vi "PicoScope4000ExampleStreaming.vi"() -> ()   [LabVIEW 2010]
doc: "This example demonstrates how to use the PicoScope Labview library to stream data from a PicoScope 4000 Series Device"
uses:
  PicoScope4000Lib/PicoScope4000AnalogChannelSettingsIEPE.ctl
  PicoScope4000Lib/PicoScope4000Buffer and Transfer Settings.ctl
panel:
  in  "Write TDMS":bool
  in  "Channel B Settings":T1={"Enabled"=FALSE, "Range"=6, "Bandwidth Limit"=0, "Coupling"=1} {"Coupling" items=["AC", "DC", "IEPE"]; "Bandwidth Limit" items=["Off", "200kHz"]; "Range" items=["10 mV", "20 mV", "50 mV", "100 mV", "200 mV", "500 mV", "1 V", "2 V", "5 V", "10 V", "20 V", "50 V ", "100 V"]}
  out "Unit Info":T2
  in  "Channel A Settings":T1={"Enabled"=TRUE, "Range"=6, "Bandwidth Limit"=0, "Coupling"=1} {"Coupling" items=["AC", "DC", "IEPE"]; "Bandwidth Limit" items=["Off", "200kHz"]; "Range" items=["10 mV", "20 mV", "50 mV", "100 mV", "200 mV", "500 mV", "1 V", "2 V", "5 V", "10 V", "20 V", "50 V ", "100 V"]}
  out "Analog Channels":cluster{i32, dbl, "Data (Volts)":dbl[]}[](graph)=[{0, 8e-09, "Data (Volts)"=[]}, {0, 8e-09, "Data (Volts)"=[]}, {0, 8e-09, "Data (Volts)"=[]}, {0, 8e-09, "Data (Volts)"=[]}, {0, 8e-09, "Data (Volts)"=[]}, {0, 8e-09, "Data (Volts)"=[]}, {0, 8e-09, "Data (Volts)"=[]}, {0, 8e-09, "Data (Volts)"=[]}]
  out "Raw Sample Interval (sec)":dbl format="%#.5p"
  out "Max ADC value":i16
  out "Chunk time(ms)":u32
  out "Elapsed time":dbl
  in  "Data file":path=path "PicoScope4000aExampleStreaming Data"
  out "size(s)":i32
  out "Queue depth":i32(graph)
  out "queue depth":i32
  in  "Buffer and Transfer Settings":T3={"startIndex"=0, "Samples"=1000000, "Down Sample Ratio"=1, "Down-Sample Mode"=0} {"Down-Sample Mode" items=["None", "Aggregate", "Average"]; "Down Sample Ratio" step=1; "Samples" format="%_6p"}
  out "TriggeredAt (In Buffer)":u32 format="%#.6p"
  out "TriggeredAt (Total samples)":u32 format="%#.6p"
  in  "Acquisition Settings":T4={"Auto Stop"=TRUE, "Desired Sample Interval"=1, "Pre-trigger Samples"=0, "Post-trigger Samples"=1000000, "Down-Sample Ratio"=1, "Down-Sample Mode"=0, "Time Units"=3} {"Time Units" items=["Nanoseconds (ns)"=2, "Microseconds (us)"=3, "Milliseconds (ms)"=4, "Seconds (s)"=5]; "Down-Sample Mode" items=["None"=0, "Aggregate"=1, "Decimate"=2, "Average"=4]; "Post-trigger Samples" format="%#.6p"; "Pre-trigger Samples" format="%#_6p"}
  out "Triggered":bool
  out "DownSample Interval (sec)":dbl format="%#.5p"
  out "Total Samples":u32 format="%#.6p"
  out "Auto Stopped":bool
  in  "Serial Number":string
  in  "Open Using Serial Number":bool
  out "Number of Samples per Capture":u32 format="%#.6p"
  in  "Apply Settings":bool
  in  "stop":bool
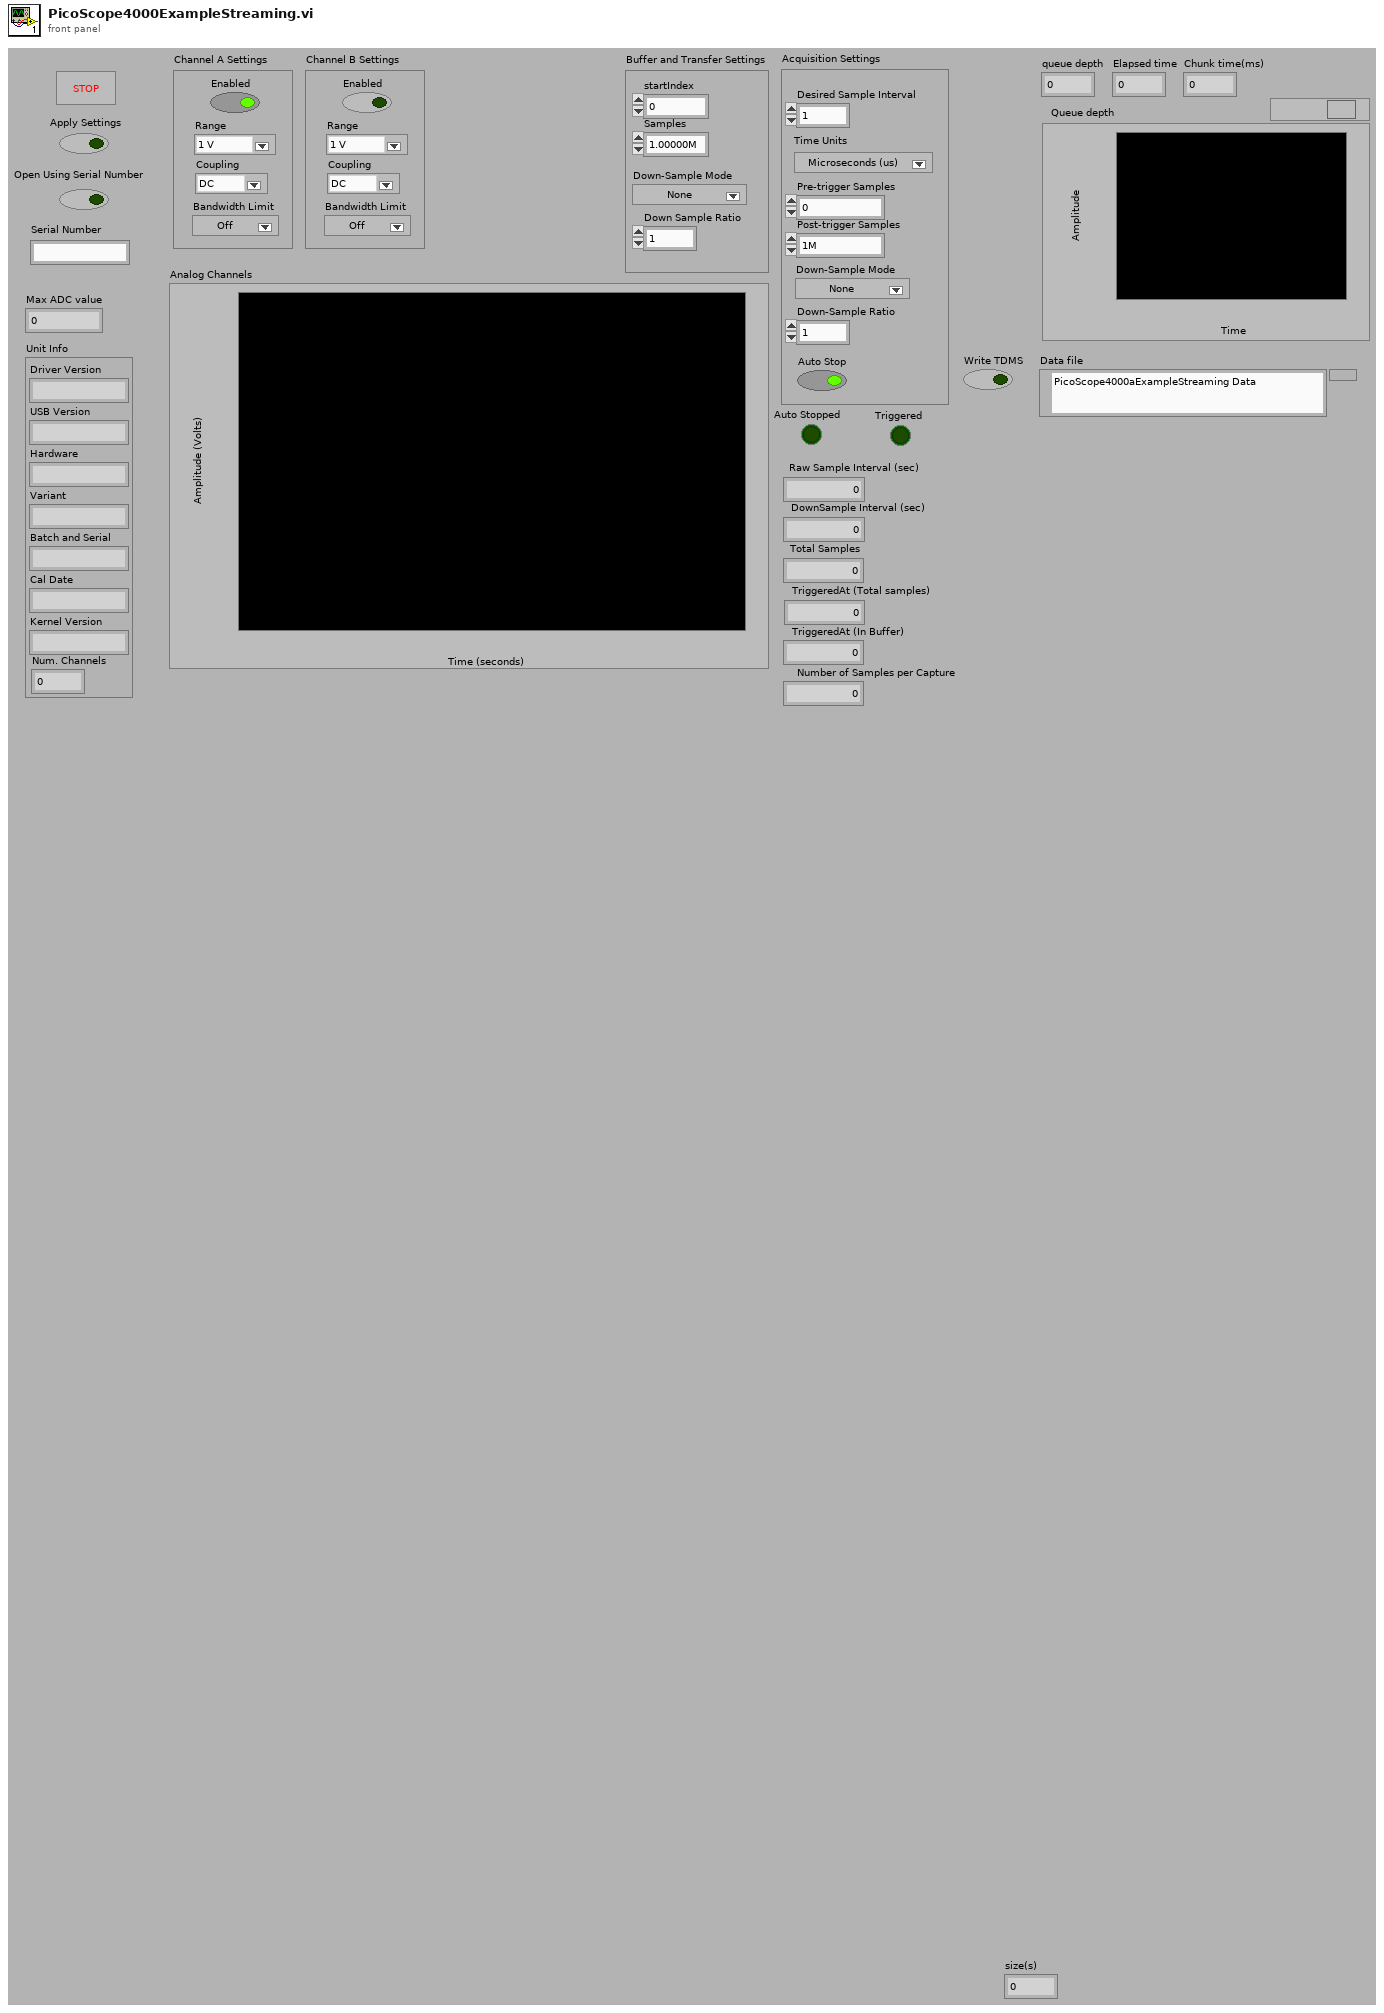
[diagram p1: front panel]
types:
  T1 = typedef "PicoScope4000AnalogChannelSettingsIEPE.ctl" = cluster{"Enabled":bool, "Range":u16, "Bandwidth Limit":i16, "Coupling":u16}
  T2 = cluster{"Driver Version":string, "USB Version":string, "Hardware":string, "Variant":string, "Batch and Serial":string, "Cal Date":string, "Kernel Version":string, "Num. Channels":i16}
  T3 = typedef "PicoScope4000Buffer and Transfer Settings.ctl" = cluster{"startIndex":u64, "Samples":u64, "Down Sample Ratio":u64, "Down-Sample Mode":u32}
  T4 = cluster{"Auto Stop":bool, "Desired Sample Interval":u32, "Pre-trigger Samples":u32, "Post-trigger Samples":u32, "Down-Sample Ratio":u32, "Down-Sample Mode":i32, "Time Units":u32}
  T5 = enum16{"open", "open or create", "create or replace", "create", "open (read-only)"}
  T6 = cluster{"Channel A Buffer":i16[], "Channel B Buffer":i16[], "Channel C Buffer":i16[], "Channel D Buffer":i16[], "Channel E Buffer":i16[], "Channel F Buffer":i16[], "Channel G Buffer":i16[], "Channel H Buffer":i16[], "Port 0":i16[], "Port 1":i16[]}
  T7 = cluster{i32, "DownSample Interval (sec)":dbl, "Data":dbl[]}
  T8 = cluster{i32, "DownSample Interval (sec)":dbl, "Data":dbl[]}[]
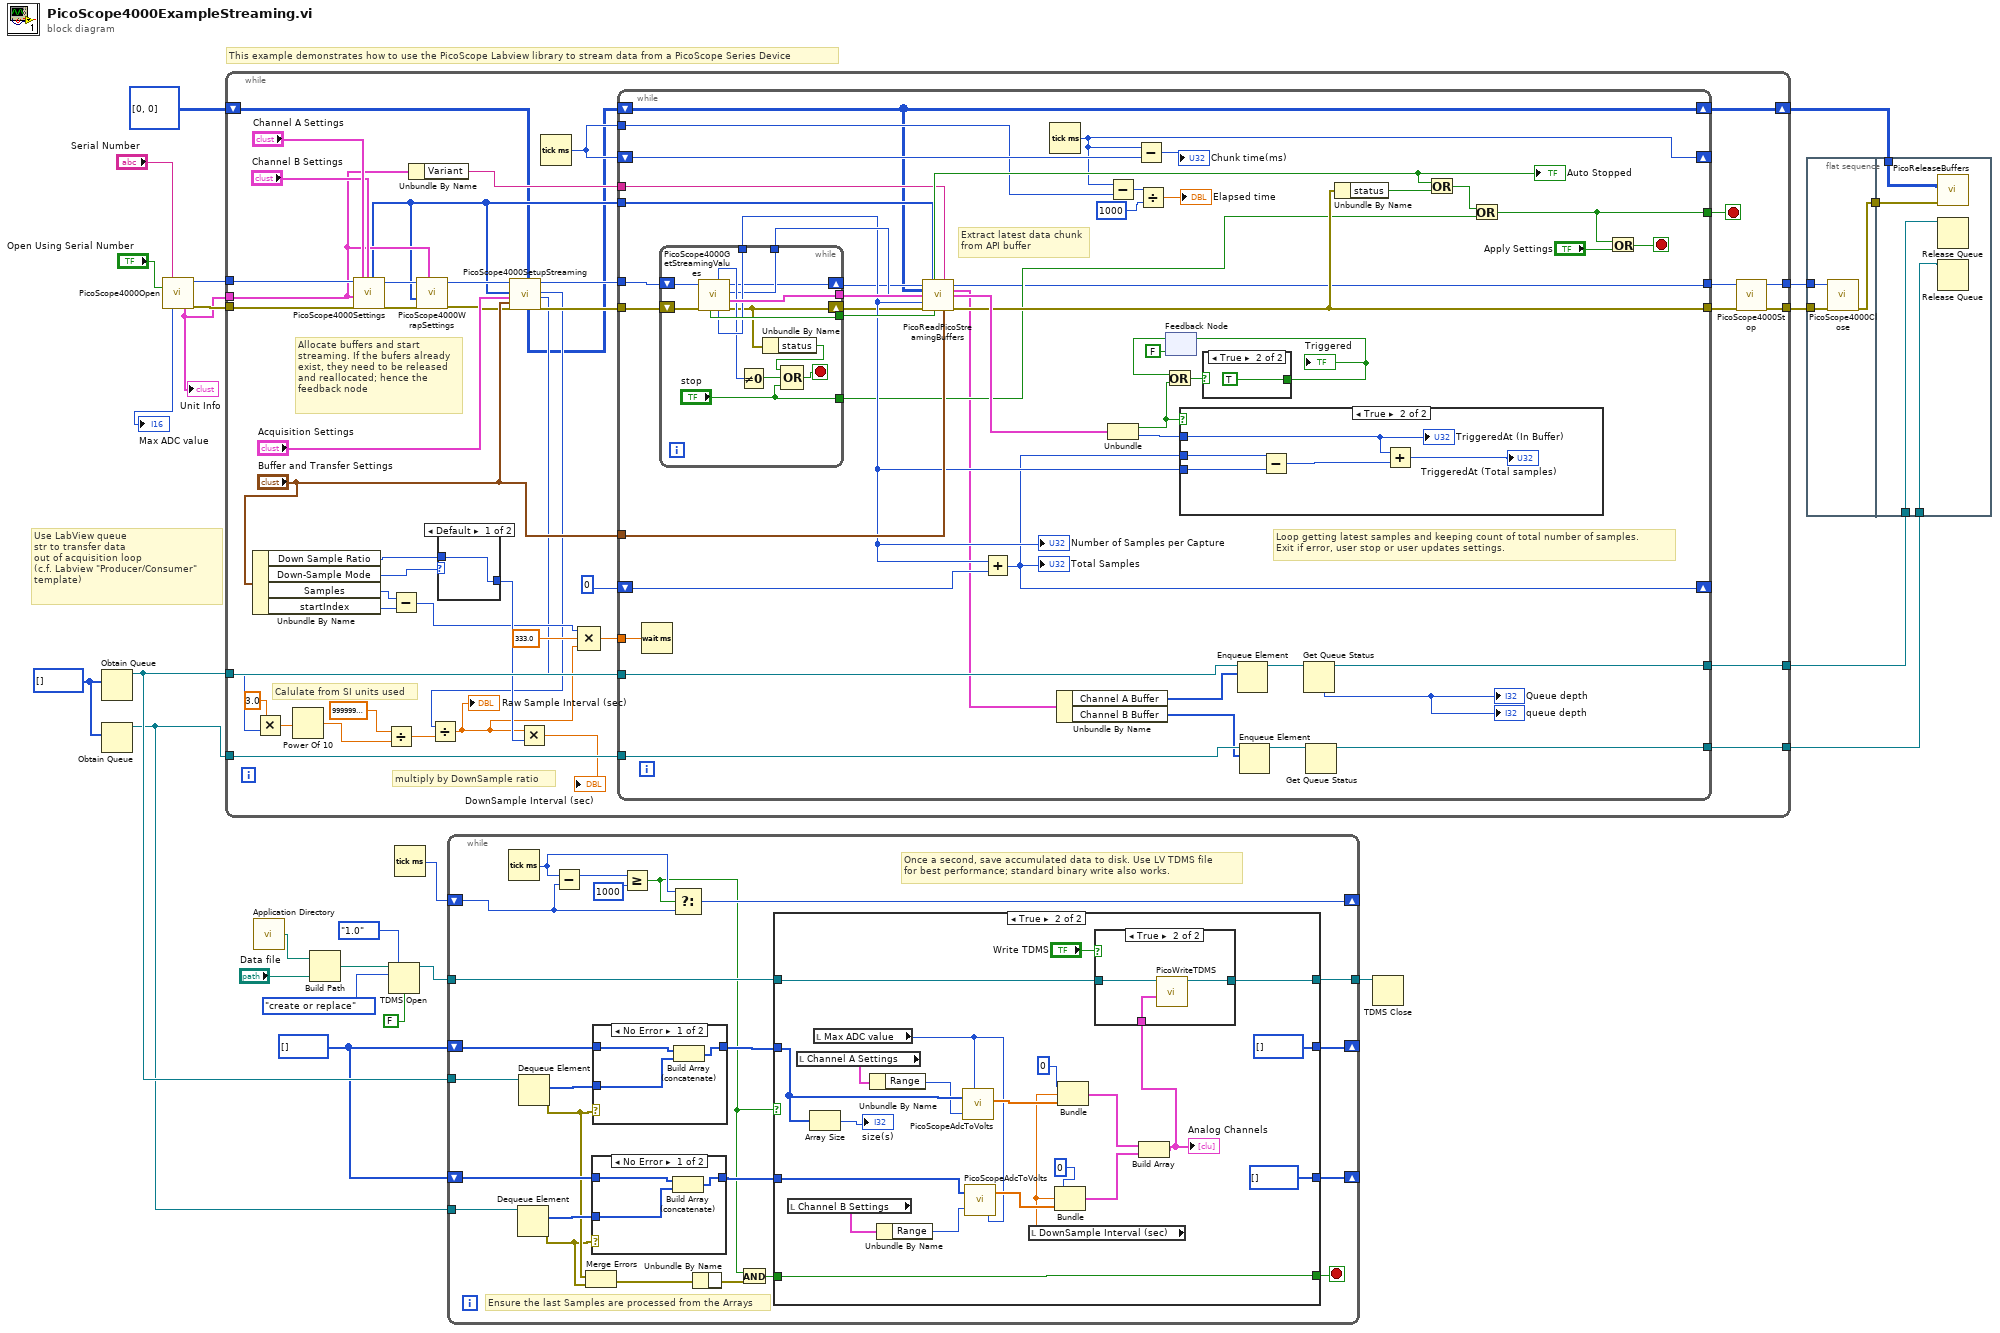
[diagram p0: block diagram]
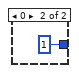
[diagram p6: hidden frame]
diagram:
  w14 = i16[] [] ("History Data")
  w17 = i16[] [] ("History Data")
  # "Use LabView queue\nstr to transfer data\nout of acquisition loop\n(c.f. Labview \"Producer/Consumer\"\ntemplate)"
  # "This example demonstrates how to use the PicoScope Labview library to stream data from a PicoScope Series Device"
  n1 = Obtain Queue(element data type=w17) -> (queue out=w26:refnum<queue>)  [unwired: 4 in, 2 out]
  n2 = Obtain Queue(element data type=w17) -> (queue out=w15:refnum<queue>)  [unwired: 4 in, 2 out]
  n3 = call "PicoScope4000Open.vi"("Serial Number"="Serial Number", "Use Serial Number"="Open Using Serial Number") -> ("handle"=w7:i16, "Max ADC value"=→"Max ADC value":i16, "Unit Info"=w5:T2, "error out"=w6:errorcluster)  [unwired: 10 in]
  "Unit Info" <- w5
  n4 = while {
    tunnel: [w60] -> w25
    tunnel: w7 -> [w71]
    tunnel: [w66] -> w24
    tunnel: w26 -> [w65]
    tunnel: [w64] -> w16
    tunnel: w15 -> [w63]
    tunnel: w6 -> [w45]
    tunnel: w5 -> [w41]
    tunnel: [w30] -> w4
    shift-right: [w27] -> w1
    shift-left: u64[][] [[0], [0]] ("Pointer array") -> [w29]
    stop <- w72 stop-if-true
    # "multiply by DownSample ratio"
    # "Calulate from SI units used"
    # "Allocate buffers and start\nstreaming. If the bufers already\nexist, they need to be released\nand reallocated; hence the\nfeedback node"
    n5 = Unbundle By Name("Buffer and Transfer Settings") -> ("Down Sample Ratio"=w69:u64, "Down-Sample Mode"=w70:u32, "Samples"=w51:u64, "startIndex"=w50:u64)
    n6 = call "PicoScope4000Settings.vi"("handle in"=w71, "Unit Info"=w41, "error in"=w45, "Channel A Settings"="Channel A Settings", "Channel B Settings"="Channel B Settings") -> ("Enabled array"=w34:i16[], "handle out"=w38:i16, "error out"=w39:errorcluster)  [unwired: 12 in]
    n7 = Subtract(x=w51, y=w50) -> (x-y=w49:u64)
    n8 = Unbundle By Name(w41) -> ("Variant"=w42:string)
    n9 = call "PicoScope4000WrapSettings.vi"("Unit Info"=w41, "error in (no error)"=w39, "Enabled array"=w34, "Handle In"=w38) -> ("error out"=w33:errorcluster, "Handle Out"=w37:i16)  [unwired: 6 in]
    n10 = case shown="Default" w70 {
      tunnel: [w73 u32 1 ("Down-Sample Ratio")] -> w53
      tunnel: w69 -> [w73 _]
      frame Default {
      }
      frame 0 {
      }
    }
    n11 = call "PicoScope4000SetupStreaming.vi"("handle in"=w37, "enabled array"=w34, "Acquisition Settings"="Acquisition Settings", "Buffer and Transfer Settings"="Buffer and Transfer Settings", "error in"=w33, "Pointers In"=w29) -> ("Pointer array"=w28:u64[][], "handle out"=w36:i16, "Sample Interval"=w32:u32, "sampleIntervalTimeUnits"=w31:u32, "error out"=w35:errorcluster)  [unwired: 9 in]
    n12 = Multiply(x=3.0, y=w31) -> (x*y=w58:dbl)
    n13 = Power Of 10(x=w58) -> (10^x=w57:dbl)
    n14 = Divide(x=sgl 1000000000000000.0 ("y"), y=w57) -> (x/y=w54:dbl)
    n15 = Divide(x=w32, y=w54) -> (x/y=w46:dbl)
    "Raw Sample Interval (sec)" <- w46
    n16 = Multiply(x=w46, y=w53) -> (x*y=→"DownSample Interval (sec)":dbl)
    n17 = Tick Count (ms)() -> (millisecond timer value=w59:u32)
    n18 = Compound Arithmetic op=MULTIPLY(w49, 333.0 ("value"), w46) -> (w52:dbl)
    n19 = while {
      tunnel: [w77] -> w61
      tunnel: [w118] -> w72
      tunnel: w35 -> [w106]
      tunnel: w36 -> [w105]
      tunnel: [w103] -> w62
      tunnel: "Buffer and Transfer Settings" -> [w104]
      tunnel: w34 -> [w102]
      tunnel: [w100] -> w66
      tunnel: w65 -> [w98]
      shift-right: [w93] -> _
      shift-left: w59 -> [w94]
      tunnel: w42 -> [w88]
      tunnel: [w86] -> w64
      tunnel: w63 -> [w85]
      tunnel: w59 -> [w82]
      tunnel: w52 -> [w81]
      shift-right: [w79] -> _
      shift-left: u32 0 -> [w80]
      shift-right: [w75] -> w27
      shift-left: w28 -> [w75]
      stop <- w117 stop-if-true
      # "Loop getting latest samples and keeping count of total number of samples. \nExit if error, user stop or user updates settings."
      # "Extract latest data chunk\nfrom API buffer"
      n20 = Wait (ms)(milliseconds to wait=w81) -> ()  [unwired: 1 out]
      n21 = while {
        tunnel: [w132] -> w116
        tunnel: [w131] -> w113
        tunnel: [w124] -> w90
        tunnel: [w130] -> w89
        shift-right: [w120] -> w78
        shift-left: w106 -> [w121]
        shift-right: [w122] -> w77
        shift-left: w105 -> [w123]
        tunnel: ["stop"] -> w83
        stop <- w126 stop-if-true
        n22 = call "PicoScope4000GetStreamingValues.vi"("error in"=w121, "handle in"=w123) -> ("error out"=w120:errorcluster, "Trigger"=w132:cluster{bool, "triggeredAt (Total samples)":u32}, "Start Index in Driver Buffer"=w124:u32, "handle out"=w122:i16, "Number of Samples"=w130:u32, "ready"=w129:i16, "Auto Stopped"=w131:bool)  [unwired: 3 in]
        n23 = Not Equal To 0?(x=w129) -> (x != 0?=w127:bool)
        n24 = Unbundle By Name(w120) -> ("status"=w128:bool)
        n25 = Compound Arithmetic op=OR(w128, w127, "stop") -> (w126:bool)
      }
      "Number of Samples per Capture" <- w89
      "Auto Stopped" <- w113
      n26 = call "PicoReadPicoStreamingBuffers.vi"("enabled array"=w102, "Buffer and Transfer Settings"=w104, "Variant"=w88, "Pointer array"=w75, "Offset Index"=w90, "Number of Samples"=w89, "error in (no error)"=w78) -> ("Buffers (Max or non-aggregated)"=w76:T6, "error out"=w103:errorcluster)  [unwired: 6 in, 1 out]
      n27 = Add(x=w89, y=w80) -> (x+y=w79:u32)
      "Total Samples" <- w79
      n28 = Tick Count (ms)() -> (millisecond timer value=w93:u32)
      n29 = Unbundle By Name(w76) -> ("Channel A Buffer"=w91:i16[], "Channel B Buffer"=w84:i16[])
      n30 = Subtract(x=w93, y=w82) -> (x-y=w97:u32)
      n31 = Unbundle(w116) -> (w108:bool, "triggeredAt (Total samples)"=w107:u32)
      n32 = Subtract(x=w93, y=w94) -> (x-y=→"Chunk time(ms)":u32)
      n33 = Divide(x=w97, y=u32 1000) -> (x/y=→"Elapsed time":dbl)
      n34 = feedback #1(FALSE) -> (w112:bool)
      n35 = Or(x=w112, y=w108) -> (x .or. y?=w110:bool)
      n36 = case shown="True" w108 {
        tunnel: w89 -> [_ w133]
        tunnel: w79 -> [_ w137]
        tunnel: w107 -> [_ w135]
        frame False {
        }
        frame True {
          n37 = Subtract(x=w137, y=w133) -> (x-y=w136:u32)
          n38 = Add(x=w135, y=w136) -> (x+y=→"TriggeredAt (Total samples)":u32)
          "TriggeredAt (In Buffer)" <- w135
        }
      }
      n39 = case shown="True" w110 {
        selector: w110 -> [w138 _]
        tunnel: [w138 TRUE] -> w109
        frame False {
        }
        frame True {
        }
      }
      "Triggered" <- w109
      n40 = feedback-in #1(w109) -> ()
      n41 = Enqueue Element(queue=w98, element=w91) -> (queue out=w99:refnum<queue>)  [unwired: 2 in, 2 out]
      n42 = Enqueue Element(queue=w85, element=w84) -> (queue out=w87:refnum<queue>)  [unwired: 2 in, 2 out]
      n43 = Get Queue Status(queue=w99) -> (queue out=w100:refnum<queue>, # elements in queue=→"queue depth" →"Queue depth":i32)  [unwired: 2 in, 6 out]
      n44 = Get Queue Status(queue=w87) -> (queue out=w86:refnum<queue>)  [unwired: 2 in, 7 out]
      n45 = Unbundle By Name(w103) -> ("status"=w115:bool)
      n46 = Or(x=w113, y=w115) -> (x .or. y?=w114:bool)
      n47 = Or(x=w114, y=w83) -> (x .or. y?=w118:bool)
      n48 = Or(x=w118, y="Apply Settings") -> (x .or. y?=w117:bool)
    }
    n49 = call "PicoScope4000Stop.vi"("error in (no error)"=w62, "handle in"=w61) -> ("error out"=w30:errorcluster, "handle out"=w60:i16)  [unwired: 8 in]
  }
  n50 = call <vilib>:"Application Directory.vi"() -> ("Application Directory"=w11:path)
  n51 = Build Path(base path=w11, name or relative path="Data file") -> (appended path=w12:path)
  n52 = TDMS Open(6:FALSE ("disable buffering? (T)"), 7:enum16{"1.0", "2.0"}."1.0" ("file format version (2.0)"), 10:T5."create or replace" ("operation (0:open)"), 11:w12) -> (3:w21:refnum<k34>)  [unwired: 2 in, 1 out]
  n53 = Tick Count (ms)() -> (millisecond timer value=w23:u32)
  n54 = while {
    tunnel: w26 -> [w162]
    shift-right: [w154] -> _
    shift-left: w14 -> [w161]
    shift-right: [w156] -> _
    shift-left: w23 -> [w157]
    tunnel: w21 -> [w153]
    tunnel: [w152] -> w20
    tunnel: w15 -> [w150]
    shift-right: [w147] -> _
    shift-left: w14 -> [w149]
    stop <- w144 stop-if-true
    # "Ensure the last Samples are processed from the Arrays"
    # "Once a second, save accumulated data to disk. Use LV TDMS file\nfor best performance; standard binary write also works."
    n55 = Tick Count (ms)() -> (millisecond timer value=w158:u32)
    n56 = Dequeue Element(queue=w150) -> (element=w151:i16[], error out=w145:errorcluster)  [unwired: 2 in, 2 out]
    n57 = Dequeue Element(queue=w162) -> (element=w163:i16[], error out=w146:errorcluster)  [unwired: 2 in, 2 out]
    n58 = Subtract(x=w158, y=w157) -> (x-y=w160:u32)
    n59 = Merge Errors(w146, w145) -> (w143:errorcluster)
    n60 = case shown="No Error" w145 {
      tunnel: w149 -> [w166 w167]
      tunnel: [w165 w167] -> w148
      tunnel: w151 -> [w164 _]
      frame No Error {
        n61 = Build Array (concatenate)(w166, w164) -> (w165:i16[])
      }
      frame Error {
      }
    }
    n62 = case shown="No Error" w146 {
      tunnel: w161 -> [w200 w201]
      tunnel: [w199 w201] -> w155
      tunnel: w163 -> [w198 _]
      frame No Error {
        n63 = Build Array (concatenate)(w200, w198) -> (w199:i16[])
      }
      frame Error {
      }
    }
    n64 = Greater Or Equal?(x=w160, y=u32 1000) -> (x >= y?=w142:bool)
    n65 = Select(t=w158, s=w142, f=w157) -> (s? t:f=w156:u32)
    n66 = And(x=w142) -> (y=w140:errorcluster, x .and. y?=w141:bool)
    n67 = Unbundle By Name(w143, w140) -> ()
    n68 = case shown="True" w142 {
      tunnel: w155 -> [w171 w191]
      tunnel: [w171 i16[] [] ("History Data")] -> w154
      tunnel: w153 -> [w170 w174]
      tunnel: [w170 w175] -> w152
      tunnel: w148 -> [w169 w179]
      tunnel: [w169 i16[] [] ("History Data")] -> w147
      tunnel: [w168 w178] -> w144
      tunnel: w141 -> [w168 w178]
      frame False {
      }
      frame True {
        n69 = local read "Channel B Settings"() -> (w176:T1)
        n70 = local read "Channel A Settings"() -> (w177:T1)
        n71 = Array Size(array=w191) -> (size(s)=→"size(s)":i32)
        n72 = local read "Max ADC value"() -> (w181:i16)
        n73 = Unbundle By Name(w177) -> ("Range"=w190:u16)
        n74 = Unbundle By Name(w176) -> ("Range"=w180:u16)
        n75 = call "PicoScopeAdcToVolts.vi"("Max_adc"=w181, "Range Index"=w190, "Data"=w191) -> ("Data"=w188:dbl[])
        n76 = call "PicoScopeAdcToVolts.vi"("Max_adc"=w181, "Range Index"=w180, "Data"=w179) -> ("Data"=w186:dbl[])
        n77 = local read "DownSample Interval (sec)"() -> (w185:dbl)
        n78 = Bundle(0, "DownSample Interval (sec)"=w185, "Data"=w186) -> (w182:T7)  [unwired: 1 in]
        n79 = Bundle(0, "DownSample Interval (sec)"=w185, "Data"=w188) -> (w183:T7)  [unwired: 1 in]
        n80 = Build Array(w183, w182) -> (w172:T8)
        "Analog Channels" <- w172
        n81 = case shown="True" "Write TDMS" {
          tunnel: [w194 w197] -> w175
          tunnel: w174 -> [w194 w196]
          tunnel: w172 -> [_ w195]
          frame False {
          }
          frame True {
            n82 = call "PicoWriteTDMS.vi"("Analog Channels"=w195, "Refnum in"=w196) -> ("Refnum out"=w197:refnum<k34>)  [unwired: 8 in, 1 out]
          }
        }
      }
    }
  }
  n83 = TDMS Close(11:w20) -> ()  [unwired: 1 in, 2 out]
  n84 = flat-sequence {
    tunnel: w25 -> [w204]
    tunnel: w4 -> [w203]
    tunnel: [w202] -> w3
    tunnel: w24 -> [w208]
    tunnel: w16 -> [w207]
    tunnel: w3 -> [w206]
    tunnel: w1 -> [w205]
    frame #0 {
      n85 = call "PicoScope4000Close.vi"("error in (no error)"=w203, "handle"=w204) -> ("error out"=w202:errorcluster)  [unwired: 9 in]
    }
    frame #1 {
      n86 = call "PicoReleaseBuffers.vi"("error in (no error)"=w206, "Pointer array"=w205) -> ()  [unwired: 8 in, 2 out]
      n87 = Release Queue(queue=w208) -> ()  [unwired: 2 in, 3 out]
      n88 = Release Queue(queue=w207) -> ()  [unwired: 2 in, 3 out]
    }
  }
